vi "Single Axis motor_Psi(SubVI).vi"(0 "State=1, I":dbl, 1 "Motor=0, I":i32, 2 "Position=0, I":dbl, 3 "User Input":dbl, 4 "Motor Input":dbl, 5 "Backward":bool, 6 "Forward":bool, 7 "Step diff":dbl, 9 "Motor input_L":refnum<vi>, 11 "User input_L":refnum<vi>, 13 "Step diff_L":refnum<vi>) -> (15 "right":bool, 17 "down":bool, 18 "State Chart":i32(graph), 19 "Motor State":dbl, 20 "State=1, O":dbl, 21 "Motor=0, O":i32, 22 "Position=0, O":dbl, 23 "Real Output":dbl, 24 "Motor Position":dbl, 25 "up":bool, 26 "left":bool, 27 "Moving":bool)   [LabVIEW 2018]
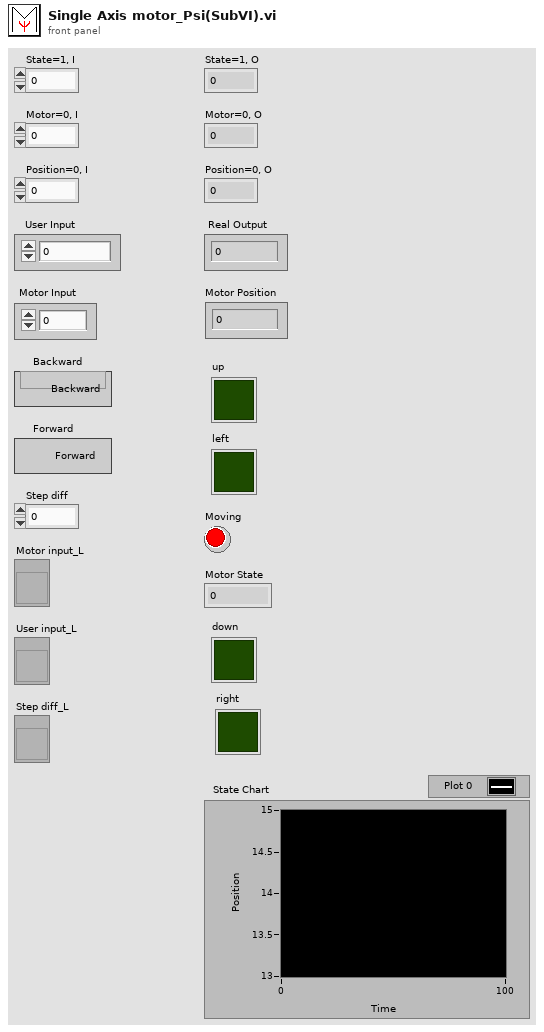
[diagram p1: front panel]
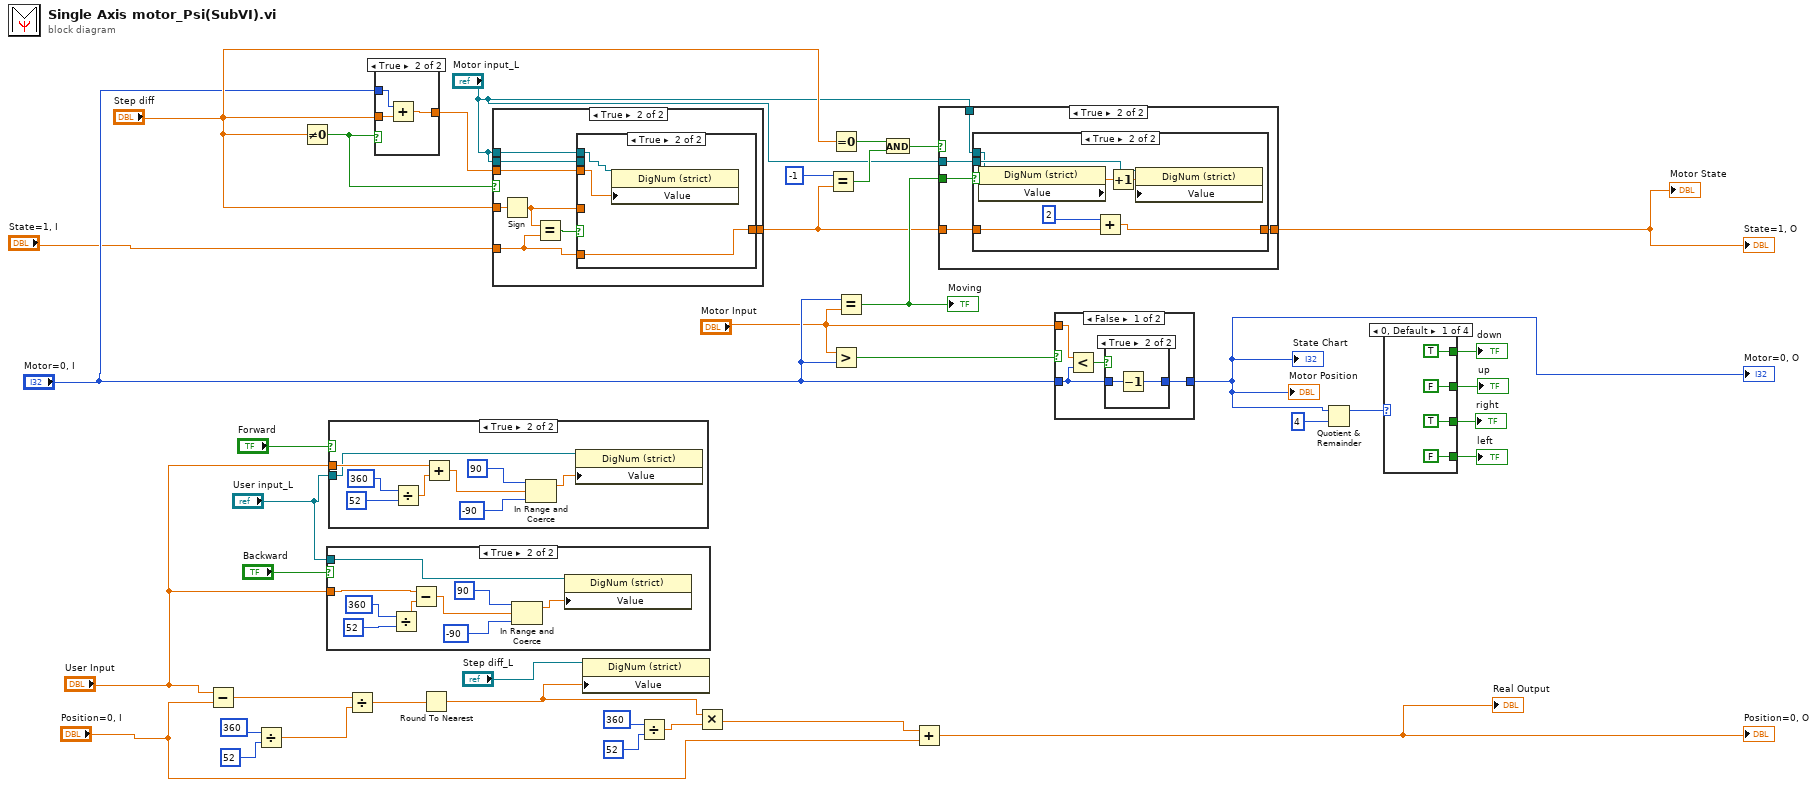
[diagram p0: block diagram]
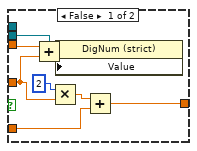
[diagram p7: hidden frame]
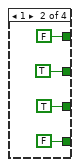
[diagram p8: hidden frame]
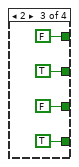
[diagram p9: hidden frame]
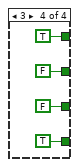
[diagram p10: hidden frame]
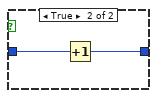
[diagram p12: hidden frame]
diagram:
  n1 = Subtract(x="User Input", y="Position=0, I") -> (x-y=w14:dbl)
  n2 = Divide(x=360, y=52) -> (x/y=w39:dbl)
  n3 = Not Equal To 0?(x="Step diff") -> (x != 0?=w8:bool)
  n4 = case shown="True" "Backward" {
    tunnel: "User Input" -> [_ w45]
    tunnel: "User input_L" -> [_ w44]
    frame False {
    }
    frame True {
      n5 = Divide(x=360, y=52) -> (x/y=w46:dbl)
      n6 = Subtract(x=w45, y=w46) -> (x-y=w41:dbl)
      n7 = In Range and Coerce(upper limit=90, x=w41, lower limit=-90) -> (coerced(x)=w40:dbl)  [unwired: 1 out]
      n8 = property class="DigNum (strict)"(reference=w44, "Value"=w40) -> ()  [unwired: 1 in, 2 out]
    }
  }
  n9 = case shown="True" "Forward" {
    tunnel: "User Input" -> [_ w54]
    tunnel: "User input_L" -> [_ w53]
    frame False {
    }
    frame True {
      n10 = Divide(x=360, y=52) -> (x/y=w55:dbl)
      n11 = Add(x=w54, y=w55) -> (x+y=w50:dbl)
      n12 = In Range and Coerce(upper limit=90, x=w50, lower limit=-90) -> (coerced(x)=w49:dbl)  [unwired: 1 out]
      n13 = property class="DigNum (strict)"(reference=w53, "Value"=w49) -> ()  [unwired: 1 in, 2 out]
    }
  }
  n14 = Divide(x=w14, y=w39) -> (x/y=w15:dbl)
  n15 = case shown="True" w8 {
    tunnel: "Motor=0, I" -> [_ w61]
    tunnel: "Step diff" -> [w58 w60]
    tunnel: [w58 w59] -> w9
    frame False {
    }
    frame True {
      n16 = Add(x=w61, y=w60) -> (x+y=w59:dbl)
    }
  }
  n17 = Round To Nearest(number=w15) -> (nearest integer value=w19:dbl)
  n18 = case shown="True" w8 {
    tunnel: [w62 w69] -> w25
    tunnel: "State=1, I" -> [w62 w68]
    tunnel: "Step diff" -> [_ w66]
    tunnel: w9 -> [_ w65]
    tunnel: "Motor input_L" -> [_ w64]
    tunnel: "Motor input_L" -> [_ w63]
    frame False {
    }
    frame True {
      n19 = Sign(1:w66) -> (0:w67:dbl)
      n20 = Equal?(x=w67, y=w68) -> (x = y?=w70:bool)
      n21 = case shown="True" w70 {
        tunnel: w67 -> [w72 _]
        tunnel: [w77 w81] -> w69
        tunnel: w68 -> [w75 w81]
        tunnel: w65 -> [w74 w80]
        tunnel: w64 -> [w71 _]
        tunnel: w63 -> [_ w79]
        frame False {
          n22 = Add(x=w74, y=w72) -> (x+y=w76:dbl)
          n23 = Multiply(x=2, y=w72) -> (x*y=w73:dbl)
          n24 = property class="DigNum (strict)"(reference=w71, "Value"=w76) -> ()  [unwired: 1 in, 2 out]
          n25 = Add(x=w73, y=w75) -> (x+y=w77:dbl)
        }
        frame True {
          n26 = property class="DigNum (strict)"(reference=w79, "Value"=w80) -> ()  [unwired: 1 in, 2 out]
        }
      }
    }
  }
  n27 = property class="DigNum (strict)"(reference="Step diff_L", "Value"=w19) -> ()  [unwired: 1 in, 2 out]
  n28 = Divide(x=360, y=52) -> (x/y=w18:dbl)
  n29 = Multiply(x=w19, y=w18) -> (x*y=w5:dbl)
  n30 = Equal?(x=-1, y=w25) -> (x = y?=w24:bool)
  n31 = Equal To 0?(x="Step diff") -> (x = 0?=w23:bool)
  n32 = Greater?(x="Motor Input", y="Motor=0, I") -> (0:w7:bool)
  n33 = Equal?(x="Motor=0, I", y="Motor Input") -> (x = y?=w35:bool)
  "Moving" <- w35
  n34 = And(x=w23, y=w24) -> (x .and. y?=w22:bool)
  n35 = Add(x=w5, y="Position=0, I") -> (x+y=→"Real Output" →"Position=0, O":dbl)
  n36 = case shown="True" w22 {
    tunnel: w25 -> [w82 w86]
    tunnel: [w82 w87] -> w21
    tunnel: w35 -> [_ w85]
    tunnel: "Motor input_L" -> [_ w84]
    tunnel: "Motor input_L" -> [_ w83]
    frame False {
    }
    frame True {
      n37 = case shown="True" w85 {
        tunnel: [w88 w93] -> w87
        tunnel: w86 -> [w88 w94]
        tunnel: w84 -> [_ w90]
        tunnel: w83 -> [_ w89]
        frame False {
        }
        frame True {
          n38 = property class="DigNum (strict)"(reference=w89) -> ("Value"=w91:dbl)  [unwired: 1 in, 2 out]
          n39 = Add(x=2, y=w94) -> (x+y=w93:dbl)
          n40 = Increment(x=w91) -> (x+1=w92:dbl)
          n41 = property class="DigNum (strict)"(reference=w90, "Value"=w92) -> ()  [unwired: 1 in, 2 out]
        }
      }
    }
  }
  "Motor State" <- w21
  "State=1, O" <- w21
  n42 = case shown="False" w7 {
    tunnel: "Motor=0, I" -> [w97 w104]
    tunnel: [w96 w103] -> w20
    tunnel: "Motor Input" -> [w99 _]
    frame False {
      n43 = Less?(x=w99, y=w97) -> (x < y?=w98:bool)
      n44 = case shown="True" w98 {
        tunnel: w97 -> [w100 w102]
        tunnel: [w100 w101] -> w96
        frame False {
        }
        frame True {
          n45 = Decrement(x=w102) -> (x-1=w101:i32)
        }
      }
    }
    frame True {
      n46 = Increment(x=w104) -> (x+1=w103:i32)
    }
  }
  "State Chart" <- w20
  "Motor Position" <- w20
  "Motor=0, O" <- w20
  n47 = Quotient & Remainder(x=w20, y=4) -> (x-y*floor(x/y)=w27:i32)  [unwired: 1 out]
  n48 = case shown="0, Default" w27 {
    tunnel: [FALSE FALSE TRUE TRUE] -> w31
    tunnel: [TRUE TRUE FALSE FALSE] -> w30
    tunnel: [FALSE TRUE TRUE FALSE] -> w29
    tunnel: [TRUE FALSE FALSE TRUE] -> w28
    frame 0, Default {
    }
    frame 1 {
    }
    frame 2 {
    }
    frame 3 {
    }
  }
  "up" <- w29
  "down" <- w28
  "right" <- w30
  "left" <- w31
